vi "G-Read-Uart_config.vi"(8 "error in (no error)":errorcluster caption="错误输入（无错误）", 11 "G-Uart-Class 输入":refnum<class "G-Uart-Class.lvclass">) -> (0 "error out":errorcluster caption="错误输出", 2 "data":string[][](array[string]), 3 "G-Uart-Class 输出":refnum<class "G-Uart-Class.lvclass">)   [LabVIEW 2025, in "G-Uart-Class.lvclass"]
uses:
  G-Uart-Class.lvclass
  <vilib>/Utility/NIReport.llb/Report Type.ctl
  <vilib>/addons/_office/excel.llb/Excel Get Data ([str]).vi
  <vilib>/Utility/NIReport.llb/NI_report.lvclass
  <vilib>/Utility/NIReport.llb/NI_ReportGenerationCore.lvlib
  <vilib>/Utility/NIReport.llb/Excel/NI_Excel.lvclass
  <vilib>/addons/_office/NI_ReportGenerationToolkit.lvlib
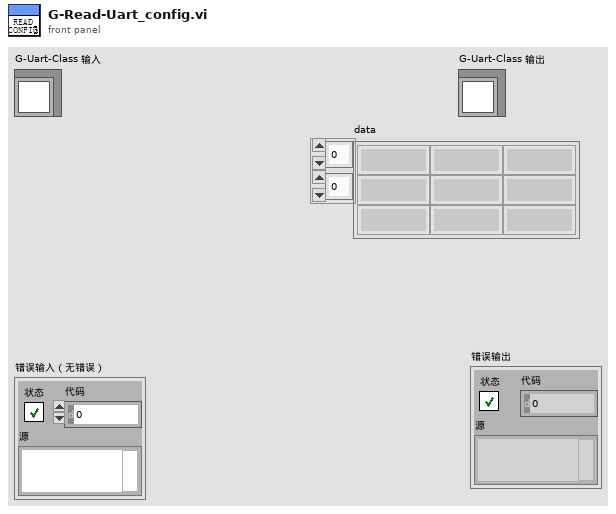
[diagram p1: front panel]
types:
  T1 = typedef "NI_ReportGenerationCore.lvlib/Report Type.ctl" = enum16{"HTML", "Word", "Excel"}
  T2 = enum16{"maximized", "minimized", "normal", "no change"}
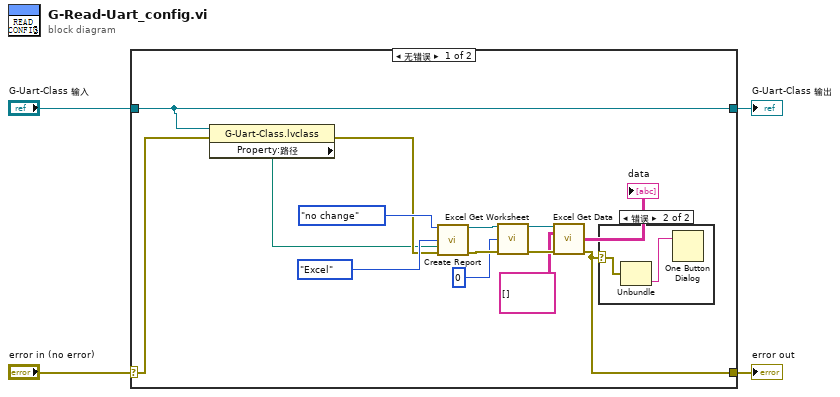
[diagram p0: block diagram]
diagram:
  n1 = case shown="无错误" "error in (no error)" {
    selector: "error in (no error)" -> [w17 w22]
    tunnel: [w7 w22] -> w3
    tunnel: [w18 w21] -> w1
    tunnel: "G-Uart-Class 输入" -> [w18 w21]
    frame No Error {
      n2 = property class="G-Uart-Class.lvclass"(reference=w18, error in=w17) -> (error out=w8:errorcluster, "Property:路径"=w5:path)  [unwired: 1 out]
      n3 = call <vilib>:"Create Report.vi"("window state (normal)"=T2."no change", "report type"=Report_Type."Excel", "template (empty)"=w5, "error in (no error)"=w8) -> ("report out"=w14:refnum<class "NI_report.lvclass">, "error out"=w13:errorcluster)  [unwired: 10 in]
      n4 = call <vilib>:"Excel Get Worksheet.vi"("report in"=w14, "worksheet index (0)"=0, "error in (no error)"=w13) -> ("report out"=w11:refnum<class "NI_report.lvclass">, "error out"=w10:errorcluster)  [unwired: 11 in]
      n5 = call-poly <vilib>:"Excel Get Data.vi"("report in"=w11, "data type"=string[][] [], "error in (no error)"=w10) -> ("data"=→"data":string[][], "error out"=w7:errorcluster)  [unwired: 10 in, 1 out]
      n6 = case shown="错误" w7 {
        selector: w7 -> [_ w20]
        frame No Error {
        }
        frame Error {
          n7 = Unbundle(w20) -> ("source"=w19:string)  [unwired: 2 out]
          n8 = One Button Dialog(message=w19) -> ()  [unwired: 1 in, 1 out]
        }
      }
    }
    frame Error {
    }
  }
  "error out" <- w3
  "G-Uart-Class 输出" <- w1
